vi "CSE ISP - Find data for help.vi"(10 "position":i32, 11 "script":string) -> (0 "identifier found":string, 1 "name for help":string, 2 "type for menu":string, 3 "name for menu":string)   [LabVIEW 2021]
doc: "::: CalcExpress Toolkit :::\nCopyright (c) 2000-2026 Konstantin Shifershteyn. All rights reserved."
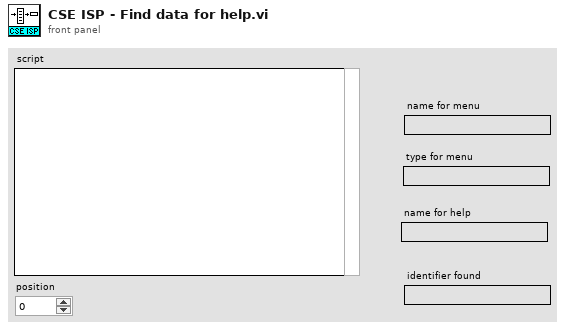
[diagram p1: front panel]
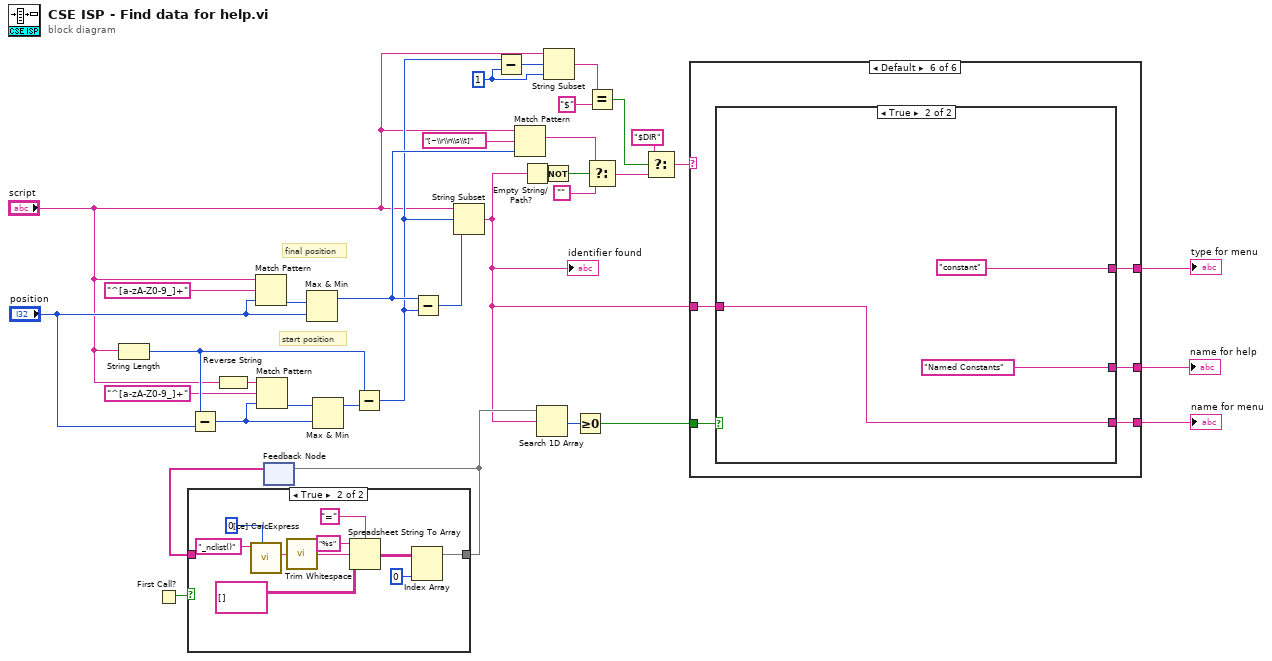
[diagram p0: block diagram]
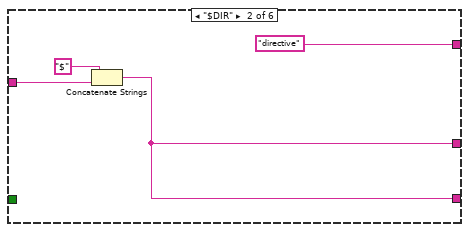
[diagram p4: hidden frame]
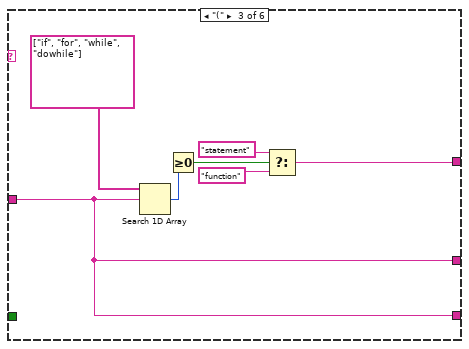
[diagram p5: hidden frame]
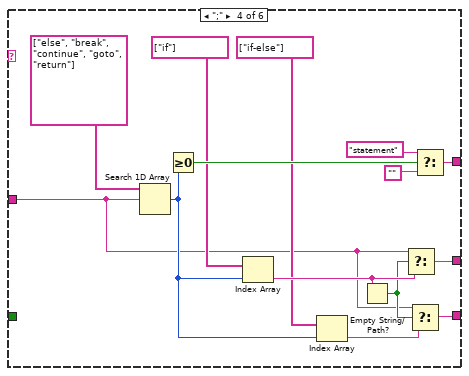
[diagram p6: hidden frame]
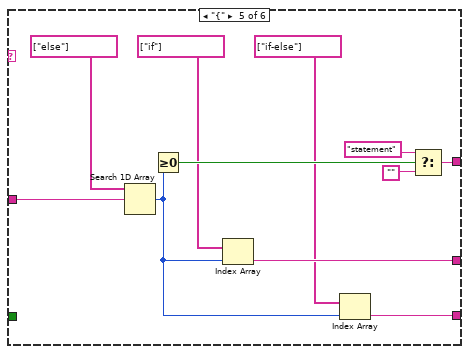
[diagram p7: hidden frame]
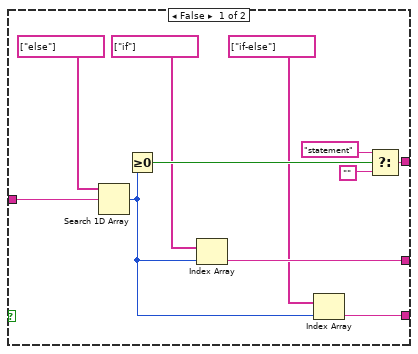
[diagram p8: hidden frame]
diagram:
  w14 = 1 ("y")
  # "start position"
  # "final position"
  n1 = String Length(string="script") -> (length=w34:i32)
  n2 = First Call?() -> (First Call?: T/F=w6:bool)
  n3 = Subtract(x=w34, y="position") -> (x-y=w32:i32)
  n4 = Reverse String(1:"script") -> (0:w29:string)
  n5 = Match Pattern(string="script", regular expression="^[a-zA-Z0-9_]+", offset (0)="position") -> (offset past match=w30:i32)  [unwired: 3 out]
  n6 = Match Pattern(string=w29, regular expression="^[a-zA-Z0-9_]+", offset (0)=w32) -> (offset past match=w31:i32)  [unwired: 3 out]
  n7 = feedback #1() -> (w5:string[])  [unwired: 1 in]
  n8 = case shown="True" w6 {
    tunnel: [w36 w37] -> w4
    tunnel: w5 -> [w36 _]
    frame False {
    }
    frame True {
      n9 = call "[ce] CalcExpress.vi"("VC Handle"=0, "expression"="_nclist()") -> ("string value"=w45:string)  [unwired: 4 in, 3 out]
      n10 = call <vilib>:"Trim Whitespace.vi"("string"=w45) -> ("trimmed string"=w40:string)  [unwired: 1 in]
      n11 = Spreadsheet String To Array(delimiter (Tab)="=", format string="%s", spreadsheet string=w40, array type (2D Dbl)=string[][] []) -> (array=w39:string[][])
      n12 = Index Array(array=w39, index (col)=0 ("disabled index (col)")) -> (element=w37:string[])  [unwired: 1 in]
    }
  }
  n13 = feedback-in #1(w4) -> ()
  n14 = Max & Min(x=w30, y="position") -> (max(x,y)=w25:i32)  [unwired: 1 out]
  n15 = Max & Min(x=w31, y=w32) -> (max(x,y)=w33:i32)  [unwired: 1 out]
  n16 = Subtract(x=w34, y=w33) -> (x-y=w15:i32)
  n17 = Subtract(x=w25, y=w15) -> (x-y=w35:i32)
  n18 = String Subset(string="script", offset (0)=w15, length (rest)=w35) -> (substring=w3:string)
  "identifier found" <- w3
  n19 = Subtract(x=w15, y=w14) -> (x-y=w16:i32)
  n20 = Match Pattern(string="script", regular expression="[~\\r\\n\\s\\t]", offset (0)=w25) -> (match substring=w19:string)  [unwired: 3 out]
  n21 = Empty String/Path?(string/path=w3) -> (empty?=w23:bool)
  n22 = Search 1D Array(1D array=w4, element=w3) -> (index of element=w2:i32)  [unwired: 1 in]
  n23 = Not(x=w23) -> (.not. x?=w20:bool)
  n24 = String Subset(string="script", offset (0)=w16, length (rest)=w14) -> (substring=w12:string)
  n25 = Greater Or Equal To 0?(x=w2) -> (x >= 0?=w1:bool)
  n26 = Equal?(x=w12, y="$") -> (x = y?=w9:bool)
  n27 = Select(t=w19, s=w20, f="") -> (s? t:f=w10:string)
  n28 = Select(t="$DIR", s=w9, f=w10) -> (s? t:f=w8:string)
  n29 = case shown="Default" w8 {
    tunnel: w3 -> [w47 w51 w52 w60 w82 w88]
    tunnel: [_ "directive" w53 w69 w79 w87] -> w21
    tunnel: [w47 w50 w52 w65 w76 w86] -> w18
    tunnel: [w47 w50 w52 w59 w73 w85] -> w17
    tunnel: w1 -> [_ _ _ _ _ w84]
    frame "" {
    }
    frame "$DIR" {
      n30 = Concatenate Strings("$", w51) -> (w50:string)
    }
    frame "(" {
      n31 = Search 1D Array(1D array=string[] ["if", "for", "while", "dowhile"], element=w52) -> (index of element=w57:i32)  [unwired: 1 in]
      n32 = Greater Or Equal To 0?(x=w57) -> (x >= 0?=w56:bool)
      n33 = Select(t="statement", s=w56, f="function") -> (s? t:f=w53:string)
    }
    frame ";" {
      n34 = Search 1D Array(1D array=string[] ["else", "break", "continue", "goto", "return"], element=w60) -> (index of element=w62:i32)  [unwired: 1 in]
      n35 = Greater Or Equal To 0?(x=w62) -> (x >= 0?=w71:bool)
      n36 = Index Array(array=string[] ["if"], index=w62) -> (element=w66:string)
      n37 = Index Array(array=string[] ["if-else"], index=w62) -> (element=w64:string)
      n38 = Empty String/Path?(string/path=w66) -> (empty?=w61:bool)
      n39 = Select(t=w60, s=w61, f=w66) -> (s? t:f=w65:string)
      n40 = Select(t=w60, s=w61, f=w64) -> (s? t:f=w59:string)
      n41 = Select(t="statement", s=w71, f="") -> (s? t:f=w69:string)
    }
    frame "{" {
      n42 = Search 1D Array(1D array=string[] ["else"], element=w82) -> (index of element=w74:i32)  [unwired: 1 in]
      n43 = Greater Or Equal To 0?(x=w74) -> (x >= 0?=w81:bool)
      n44 = Index Array(array=string[] ["if"], index=w74) -> (element=w76:string)
      n45 = Index Array(array=string[] ["if-else"], index=w74) -> (element=w73:string)
      n46 = Select(t="statement", s=w81, f="") -> (s? t:f=w79:string)
    }
    frame Default {
      n47 = case shown="True" w84 {
        tunnel: w88 -> [w98 w101]
        tunnel: [w95 "constant"] -> w87
        tunnel: [w92 "Named Constants"] -> w86
        tunnel: [w89 w101] -> w85
        frame False {
          n48 = Search 1D Array(1D array=string[] ["else"], element=w98) -> (index of element=w90:i32)  [unwired: 1 in]
          n49 = Greater Or Equal To 0?(x=w90) -> (x >= 0?=w97:bool)
          n50 = Index Array(array=string[] ["if"], index=w90) -> (element=w92:string)
          n51 = Index Array(array=string[] ["if-else"], index=w90) -> (element=w89:string)
          n52 = Select(t="statement", s=w97, f="") -> (s? t:f=w95:string)
        }
        frame True {
        }
      }
    }
  }
  "type for menu" <- w21
  "name for help" <- w18
  "name for menu" <- w17
